vi "AI_Score_Candidates.vi"(0 "Grid":enum8{"Empty", "Black", "White"}[][](array[ring])=[[enum."Empty", enum."Empty", enum."Empty", enum."Empty", enum."Empty", enum."Empty", enum."Empty", enum."Empty", enum."Empty", enum."Empty", enum."Empty", enum."Empty", enum."Empty", enum."Empty", enum."Empty"], [enum."Empty", enum."Empty", enum."Empty", enum."Empty", enum."Empty", enum."Empty", enum."Empty", enum."Empty", enum."Empty", enum."Empty", enum."Empty", enum."Empty", enum."Empty", enum."Empty", enum."Empty"], [enum."Empty", enum."Empty", enum."Empty", enum."Empty", enum."Empty", enum."Empty", enum."Empty", enum."Empty", enum."Empty", enum."Empty", enum."Empty", enum."Empty", enum."Empty", enum."Empty", enum."Empty"], [enum."Empty", enum."Empty", enum."Empty", enum."Empty", enum."Empty", enum."Empty", enum."Empty", enum."Empty", enum."Empty", enum."Empty", enum."Empty", enum."Empty", enum."Empty", enum."Empty", enum."Empty"], [enum."Empty", enum."Empty", enum."Empty", enum."Empty", enum."Empty", enum."Empty", enum."Empty", enum."Empty", enum."Empty", enum."Empty", enum."Empty", enum."Empty", enum."Empty", enum."Empty", enum."Empty"], [enum."Empty", enum."Empty", enum."Empty", enum."Empty", enum."Empty", enum."Empty", enum."Empty", enum."Empty", enum."Empty", enum."Empty", enum."Empty", enum."Empty", enum."Empty", enum."Empty", enum."Empty"], [enum."Empty", enum."Empty", enum."Empty", enum."Empty", enum."Empty", enum."Empty", enum."Empty", enum."Empty", enum."Empty", enum."Empty", enum."Empty", enum."Empty", enum."Empty", enum."Empty", enum."Empty"], [enum."Empty", enum."Empty", enum."Empty", enum."Empty", enum."Empty", enum."Empty", enum."Empty", enum."Empty", enum."Empty", enum."Empty", enum."Empty", enum."Empty", enum."Empty", enum."Empty", enum."Empty"], [enum."Empty", enum."Empty", enum."Empty", enum."Empty", enum."Empty", enum."Empty", enum."Empty", enum."Empty", enum."Empty", enum."Empty", enum."Empty", enum."Empty", enum."Empty", enum."Empty", enum."Empty"], [enum."Empty", enum."Empty", enum."Empty", enum."Empty", enum."Empty", enum."Empty", enum."Empty", enum."Empty", enum."Empty", enum."Empty", enum."Empty", enum."Empty", enum."Empty", enum."Empty", enum."Empty"], [enum."Empty", enum."Empty", enum."Empty", enum."Empty", enum."Empty", enum."Empty", enum."Empty", enum."Empty", enum."Empty", enum."Empty", enum."Empty", enum."Empty", enum."Empty", enum."Empty", enum."Empty"], [enum."Empty", enum."Empty", enum."Empty", enum."Empty", enum."Empty", enum."Empty", enum."Empty", enum."Empty", enum."Empty", enum."Empty", enum."Empty", enum."Empty", enum."Empty", enum."Empty", enum."Empty"], [enum."Empty", enum."Empty", enum."Empty", enum."Empty", enum."Empty", enum."Empty", enum."Empty", enum."Empty", enum."Empty", enum."Empty", enum."Empty", enum."Empty", enum."Empty", enum."Empty", enum."Empty"], [enum."Empty", enum."Empty", enum."Empty", enum."Empty", enum."Empty", enum."Empty", enum."Empty", enum."Empty", enum."Empty", enum."Empty", enum."Empty", enum."Empty", enum."Empty", enum."Empty", enum."Empty"], [enum."Empty", enum."Empty", enum."Empty", enum."Empty", enum."Empty", enum."Empty", enum."Empty", enum."Empty", enum."Empty", enum."Empty", enum."Empty", enum."Empty", enum."Empty", enum."Empty", enum."Empty"]], 5 "AI Stone":enum8{"Empty", "Black", "White"}(ring)=enum."White", 7 "Defense Weight":dbl=0.9, 9 "Noise":dbl, 11 "error in":errorcluster, 12 "Renju":bool=TRUE) -> (4 "Ranked":cluster{"Score":dbl, "Row":i32, "Col":i32}[](array[cluster]), 6 "Count":i32, 15 "error out":errorcluster)   [LabVIEW 2026]
doc: "후보 칸마다 공격 점수 + Defense Weight*수비 점수 + 중앙 보너스 + Noise*난수를 계산해 내림차순 정렬.\n렌주룰에서 AI가 흑이면 금수 칸은 -1e9로 밀어낸다."
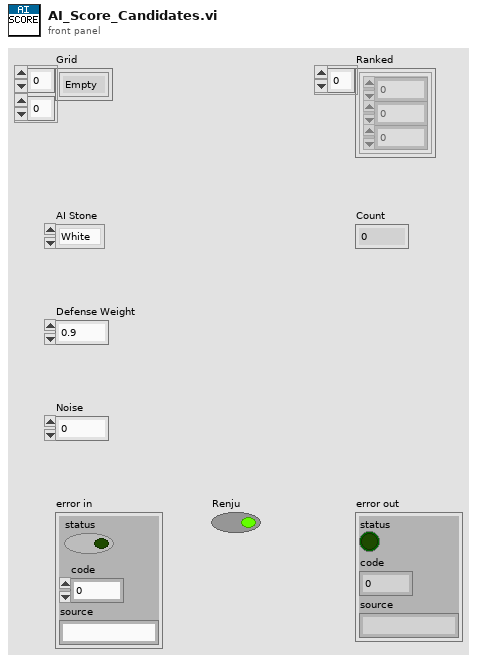
[diagram p1: front panel]
types:
  T1 = cluster{"Row":i32, "Col":i32, "Stone":enum8{"Empty", "Black", "White"}}
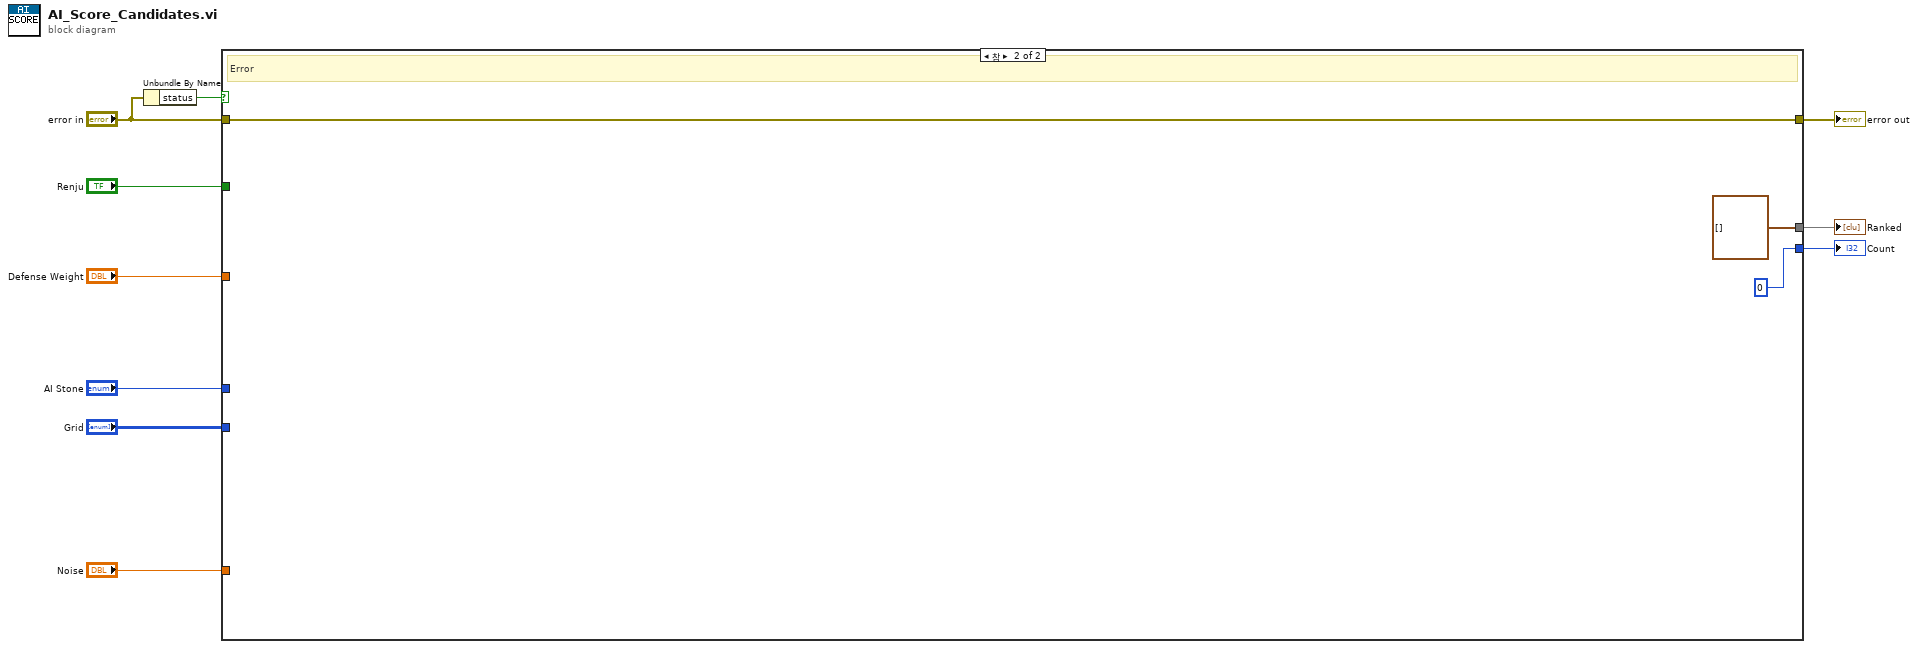
[diagram p0: block diagram]
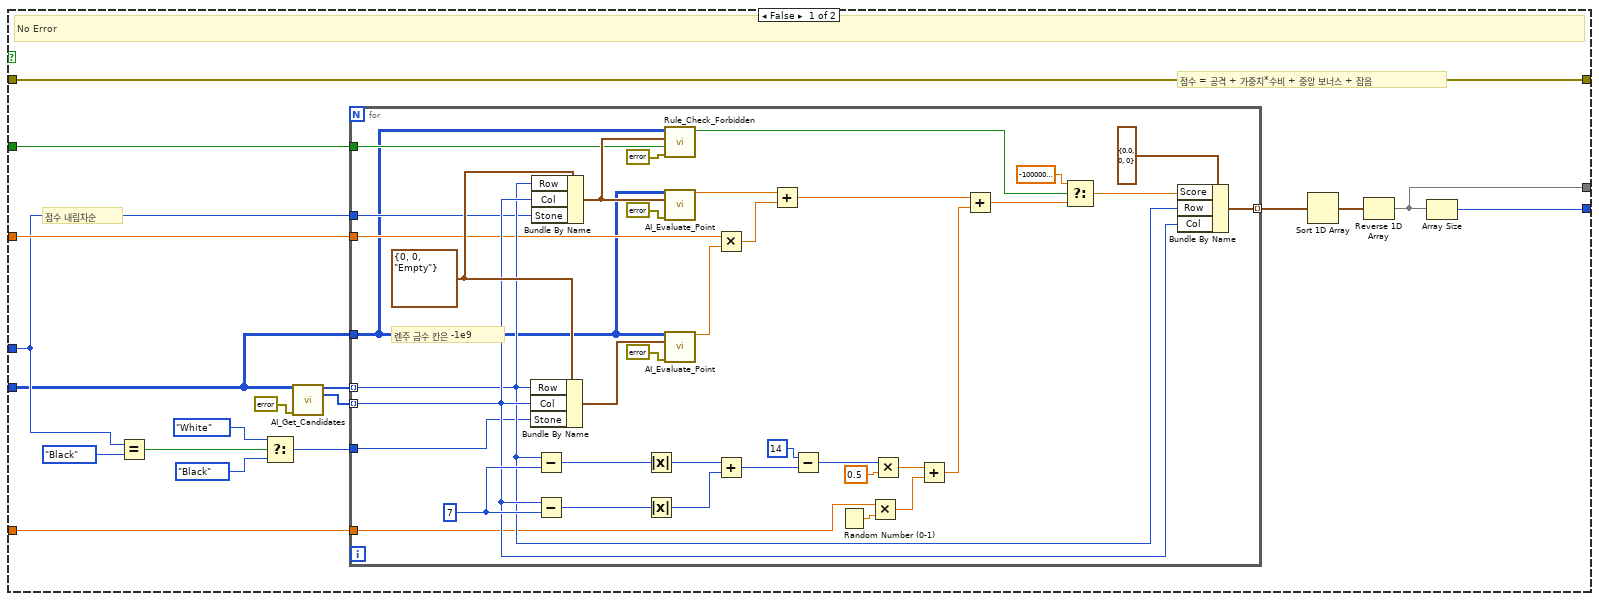
[diagram p2: hidden frame]
diagram:
  n1 = Unbundle By Name("error in") -> ("status"=w7:bool)
  n2 = case shown="참" w7 {
    tunnel: "Grid" -> [w11 _]
    tunnel: "AI Stone" -> [w12 _]
    tunnel: "Defense Weight" -> [w13 _]
    tunnel: "Noise" -> [w14 _]
    tunnel: "Renju" -> [w15 _]
    tunnel: "error in" -> [w16 w66]
    tunnel: [w16 w66] -> w10
    tunnel: [w27 cluster{"Score":dbl, "Row":i32, "Col":i32}[] []] -> w8
    tunnel: [w28 0] -> w9
    frame False {
      # "점수 내림차순"
      # "점수 = 공격 + 가중치*수비 + 중앙 보너스 + 잡음"
      # "No Error"
      n3 = Equal?(x=w12, y=enum8{"Empty", "Black", "White"}."Black") -> (x = y?=w21:bool)
      n4 = Select(t=enum8{"Empty", "Black", "White"}."White", s=w21, f=enum8{"Empty", "Black", "White"}."Black") -> (s? t:f=w24:enum8{"Empty", "Black", "White"})
      n5 = call "AI_Get_Candidates.vi"("Grid"=w11, "error in"=errorcluster {"status"=FALSE, "code"=0, "source"=""}) -> ("Rows"=w18:i32[], "Cols"=w19:i32[])  [unwired: 10 in, 2 out]
      n6 = for {
        tunnel: w11 -> [w29]
        tunnel: w12 -> [w30]
        tunnel: w13 -> [w32]
        tunnel: w14 -> [w33]
        tunnel: w15 -> [w34]
        tunnel: w18 -> [w35] mode=indexing
        tunnel: w19 -> [w36] mode=indexing
        tunnel: w24 -> [w31]
        tunnel: [w65] -> w25 mode=indexing
        w44 = 7
        w37 = T1 {"Row"=0, "Col"=0, "Stone"=enum."Empty"}
        # "렌주 금수 칸은 -1e9"
        n7 = Bundle By Name(cluster=w37, "Row"=w35, "Col"=w36, "Stone"=w31) -> (w39:T1)
        n8 = Bundle By Name(cluster=w37, "Row"=w35, "Col"=w36, "Stone"=w30) -> (w38:T1)
        n9 = Subtract(x=w35, y=w44) -> (x-y=w45:i32)
        n10 = Subtract(x=w36, y=w44) -> (x-y=w47:i32)
        n11 = Absolute Value(x=w45) -> (abs(x)=w46:i32)
        n12 = Absolute Value(x=w47) -> (abs(x)=w48:i32)
        n13 = call "Rule_Check_Forbidden.vi"("error in"=errorcluster {"status"=FALSE, "code"=0, "source"=""}, "Renju"=w34, "Move"=w38, "Grid"=w29) -> ("Forbidden?"=w61:bool)  [unwired: 5 in, 2 out]
        n14 = call "AI_Evaluate_Point.vi"("Grid"=w29, "Move"=w38, "error in"=errorcluster {"status"=FALSE, "code"=0, "source"=""}) -> ("Score"=w41:dbl)  [unwired: 11 in, 1 out]
        n15 = call "AI_Evaluate_Point.vi"("Grid"=w29, "Move"=w39, "error in"=errorcluster {"status"=FALSE, "code"=0, "source"=""}) -> ("Score"=w43:dbl)  [unwired: 11 in, 1 out]
        n16 = Multiply(x=w32, y=w43) -> (x*y=w55:dbl)
        n17 = Add(x=w46, y=w48) -> (x+y=w50:i32)
        n18 = Add(x=w41, y=w55) -> (x+y=w56:dbl)
        n19 = Subtract(x=14, y=w50) -> (x-y=w51:i32)
        n20 = Random Number (0-1)() -> (number: 0 to 1=w54:dbl)
        n21 = Multiply(x=w33, y=w54) -> (x*y=w57:dbl)
        n22 = Multiply(x=w51, y=0.5) -> (x*y=w53:dbl)
        n23 = Add(x=w53, y=w57) -> (x+y=w58:dbl)
        n24 = Add(x=w56, y=w58) -> (x+y=w59:dbl)
        n25 = Select(t=-1000000000.0, s=w61, f=w59) -> (s? t:f=w63:dbl)
        n26 = Bundle By Name(cluster=cluster{"Score":dbl, "Row":i32, "Col":i32} {"Score"=0.0, "Row"=0, "Col"=0}, "Score"=w63, "Row"=w35, "Col"=w36) -> (w65:cluster{"Score":dbl, "Row":i32, "Col":i32})
      }
      n27 = Sort 1D Array(array=w25) -> (sorted array=w26:cluster{"Score":dbl, "Row":i32, "Col":i32}[])
      n28 = Reverse 1D Array(array=w26) -> (reversed array=w27:cluster{"Score":dbl, "Row":i32, "Col":i32}[])
      n29 = Array Size(array=w27) -> (size(s)=w28:i32)
    }
    frame True {
      # "Error"
    }
  }
  "Ranked" <- w8
  "Count" <- w9
  "error out" <- w10
